vi "Cleanup.vi"(7 "Cleanup Devices? (T)":bool=TRUE, 8 "error in (no error)":errorcluster, 11 "HAL Manager in":refnum<class "HAL Manager.lvclass">) -> (0 "error out":errorcluster)   [LabVIEW 2020, in "HAL.lvlib" / "HAL Manager.lvclass"]
uses:
  HAL Manager.lvclass
  HAL Manager.lvclass/HAL Manager.ctl
  Device/Device.lvclass
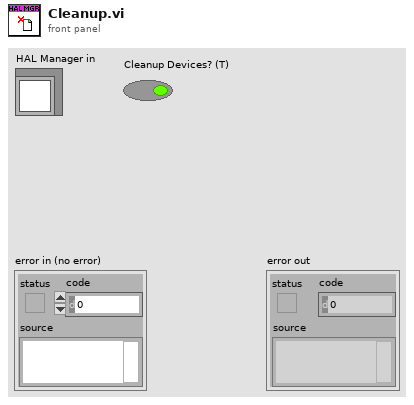
[diagram p1: front panel]
types:
  T1 = typedef "HAL.lvlib/HAL Manager.lvclass/Ref Data.ctl" = cluster{"Devices":refnum<class "Device.lvclass">[], "Type":string[], "Models":string[], "Name":string[]}
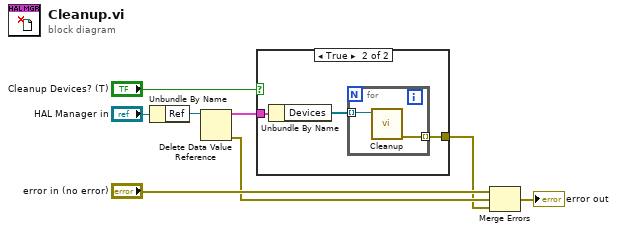
[diagram p0: block diagram]
diagram:
  n1 = Unbundle By Name("HAL Manager in") -> ("Ref"=w6:refnum<data-value>)
  n2 = Delete Data Value Reference(data value reference=w6) -> (data value=w5:T1, error out=w3:errorcluster)  [unwired: 1 in]
  n3 = case shown="True" "Cleanup Devices? (T)" {
    tunnel: w5 -> [_ w11]
    tunnel: [_ w9] -> w2
    frame False {
    }
    frame True {
      n4 = Unbundle By Name(w11) -> ("Devices"=w10:refnum<class "Device.lvclass">[])
      n5 = for {
        tunnel: w10 -> [w13] mode=indexing
        tunnel: [w12] -> w9 mode=indexing
        n6 = call "Cleanup.vi"("Device in"=w13) -> ("error out"=w12:errorcluster)  [unwired: 10 in]
      }
    }
  }
  n7 = Merge Errors("error in (no error)", w3, w2) -> (→"error out":errorcluster)
